vi "libssh2_sftp_symlink_ex.vi"(6 "target_len":u32, 7 "link_type":T1, 8 "error in (no error)":errorcluster, 9 "target in":string, 10 "path":string, 11 "sftp":T2) -> (0 "error out":errorcluster, 1 "target out":string)   [LabVIEW 2017, in "libssh2.lvlib"]
doc: "Create a symbolic link or read information about a symbolic link."
uses:
  libssh2.lvlib
  SFTP Refnum.ctl
  libssh2_sftp_symlink_type.ctl
  Acquire Session.vi
  Release Session.vi
  Not An SFTP Refnum.vi
  <vilib>/Utility/error.llb/Error Cluster From Error Code.vi
  Global Settings.vi
  Read SFTP Refnum.vi
  Read Session Refnum.vi
  <vilib>/Utility/semaphor.llb/Acquire Semaphore.vi
  <vilib>/Utility/semaphor.llb/Release Semaphore.vi
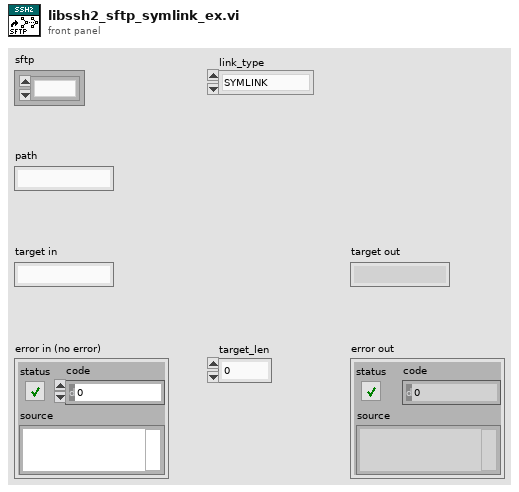
[diagram p1: front panel]
types:
  T1 = typedef "libssh2.lvlib/libssh2_sftp_symlink_type.ctl" = enum16{"SYMLINK", "READLINK", "REALPATH"}
  T2 = typedef "libssh2.lvlib/SFTP Refnum.ctl" = refnum<k1>
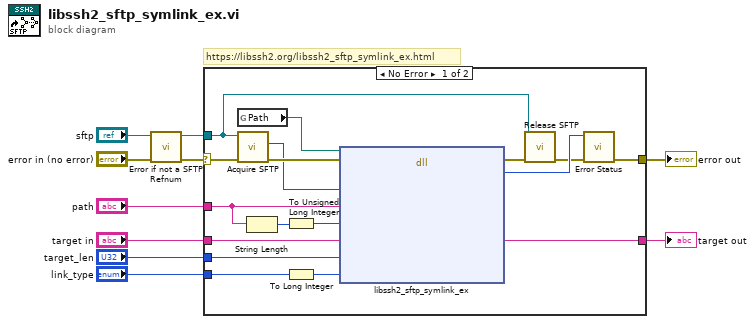
[diagram p0: block diagram]
diagram:
  # "https://libssh2.org/libssh2_sftp_symlink_ex.html"
  n1 = call "Error if not a SFTP Refnum.vi"("error in (no error)"="error in (no error)", "sftp"="sftp") -> ("error out"=w6:errorcluster, "sftp out"=w7:T2)  [unwired: 8 in]
  n2 = case shown="No Error" w6 {
    selector: w6 -> [w26 w28]
    tunnel: w7 -> [w11 _]
    tunnel: [w22 w28] -> w8
    tunnel: "path" -> [w19 _]
    tunnel: "target in" -> [w17 _]
    tunnel: "link_type" -> [w16 _]
    tunnel: [w14 _] -> w2
    tunnel: "target_len" -> [w13 _]
    frame No Error {
      n3 = global read "Global Settings.vi" "Path"() -> (w27:path)
      n4 = call "Acquire SFTP.vi"("error in (no error)"=w26, "sftp"=w11) -> ("error out"=w25:errorcluster, "LIBSSH2_SFTP*"=w24:u64)  [unwired: 8 in]
      n5 = String Length(string=w19) -> (length=w20:i32)
      n6 = To Unsigned Long Integer(number=w20) -> (unsigned 32bit integer=w18:u32)
      n7 = To Long Integer(number=w16) -> (32bit integer=w15:i32)
      n8 = dll-call lib="?" fn="libssh2_sftp_symlink_ex"(path in=w27, error in=w25, "sftp"=w24, "path"=w19, "path_len"=w18, "target"=w17, "target_len"=w13, "link_type"=w15) -> (error out=w23:errorcluster, "return value"=w21:i32, "target"=w14:string)  [unwired: 6 in, 1 out]
      n9 = call "Release SFTP.vi"("error in (no error)"=w23, "sftp"=w11) -> ("error out"=w12:errorcluster)  [unwired: 9 in]
      n10 = call "Error Status.vi"("error in (no error)"=w12, "return value"=w21) -> ("error out"=w22:errorcluster)  [unwired: 8 in, 1 out]
    }
    frame Error {
    }
  }
  "error out" <- w8
  "target out" <- w2
